vi "RemoteVI App Log Files.vi"() -> ()   [LabVIEW 2020]
doc: "Screen Log Files of RemoteVI Application Example.vi: the log files of the station (simulated - none exists on disk). Selecting a file in Log Files shows its preview and details. Delete asks in a LabVIEW dialog and removes the file from the list; Export asks for a target in the native file dialog. Runs until the notifier RemoteVI Application Example fires (the main VI quits)."
panel:
  out "Status":string
  out "Details":string
  out "Preview":dbl[][](graph)
  in  "Export":bool
  in  "Delete":bool
  in  "Log Files":i32(listbox)=-1
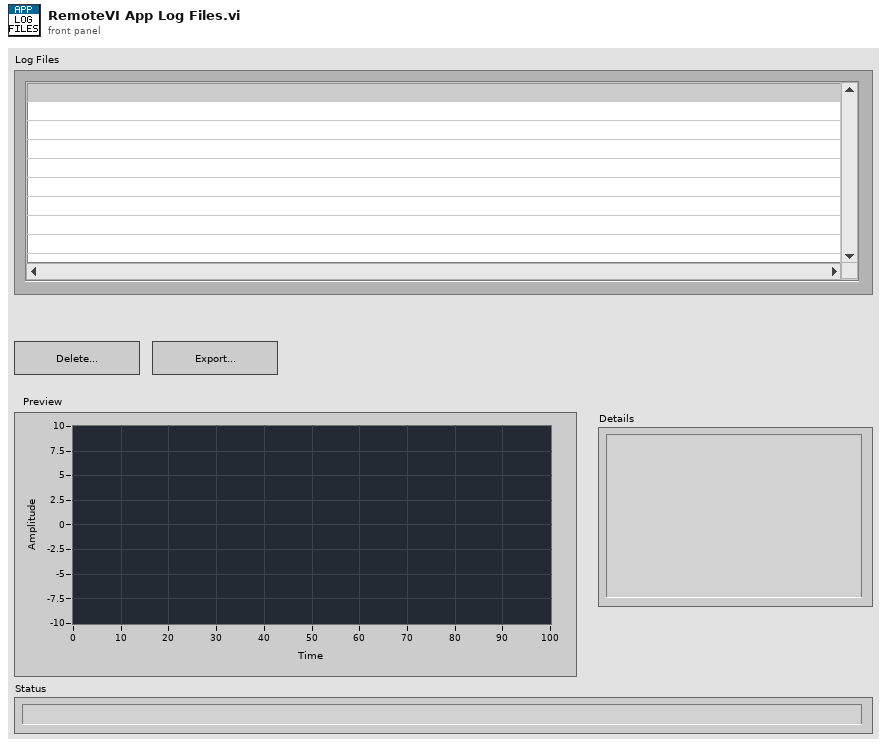
[diagram p1: front panel]
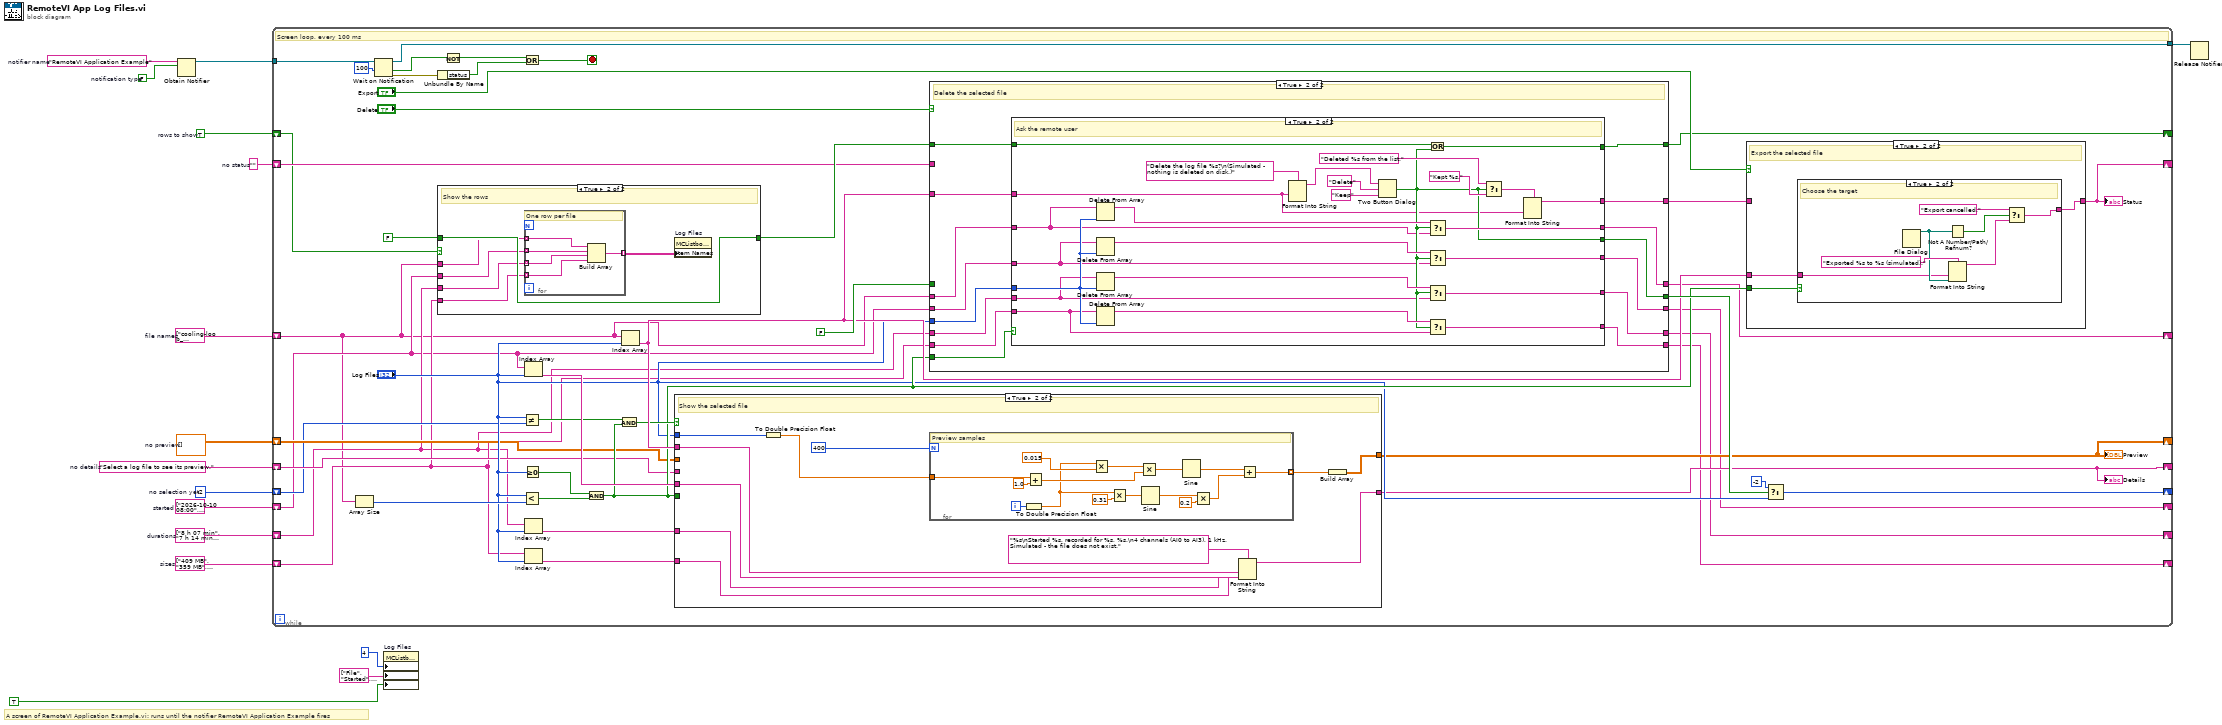
[diagram p0: block diagram]
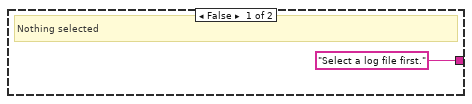
[diagram p3: hidden frame]
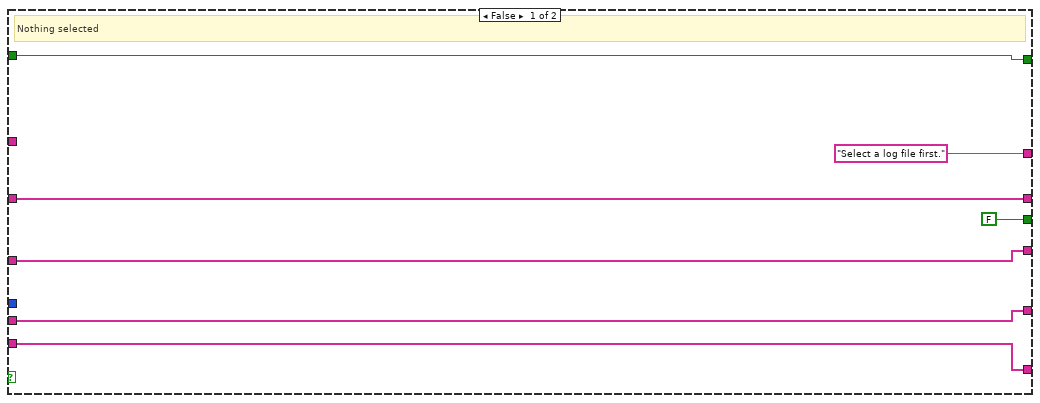
[diagram p5: hidden frame]
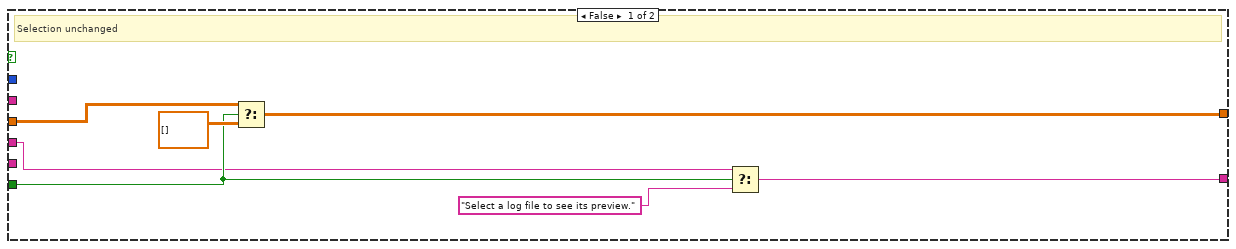
[diagram p6: hidden frame]
diagram:
  w11 = FALSE  # notification type
  w10 = "RemoteVI Application Example"  # notifier name
  w9 = ""  # no status
  w8 = "Select a log file to see its preview."  # no details
  w7 = dbl[][] []  # no preview
  w6 = -2  # no selection yet
  w5 = TRUE  # rows to show
  w4 = string[] ["409 MB", "359 MB", "411 MB", "106 MB", "413 MB", "414 MB", "364 MB", "161 MB", "417 MB", "418 MB", "419 MB", "63 MB", "421 MB", "422 MB", "423 MB", "118 MB", "374 MB", "426 MB", "427 MB", "173 MB", "429 MB"]  # sizes
  w3 = string[] ["8 h 07 min", "7 h 14 min", "8 h 21 min", "2 h 28 min", "8 h 35 min", "8 h 42 min", "7 h 49 min", "3 h 56 min", "8 h 03 min", "8 h 10 min", "8 h 17 min", "1 h 24 min", "8 h 31 min", "8 h 38 min", "8 h 45 min", "2 h 52 min", "7 h 59 min", "8 h 06 min", "8 h 13 min", "3 h 20 min", "8 h 27 min"]  # durations
  w2 = string[] ["2026-10-10 08:00", "2026-10-11 08:00", "2026-10-12 08:00", "2026-10-13 14:30", "2026-10-14 08:00", "2026-10-15 08:00", "2026-10-16 08:00", "2026-10-17 14:30", "2026-10-18 08:00", "2026-10-19 08:00", "2026-10-20 08:00", "2026-10-21 14:30", "2026-10-22 08:00", "2026-10-23 08:00", "2026-10-24 08:00", "2026-10-25 14:30", "2026-10-26 08:00", "2026-10-27 08:00", "2026-10-28 08:00", "2026-10-29 14:30", "2026-10-30 08:00"]  # started
  w1 = string[] ["cooling-loop_2026-10-10_0800.tdms", "cooling-loop_2026-10-11_0800.tdms", "cooling-loop_2026-10-12_0800.tdms", "pump-test_2026-10-13_1430.tdms", "cooling-loop_2026-10-14_0800.tdms", "cooling-loop_2026-10-15_0800.tdms", "cooling-loop_2026-10-16_0800.tdms", "pump-test_2026-10-17_1430.tdms", "cooling-loop_2026-10-18_0800.tdms", "cooling-loop_2026-10-19_0800.tdms", "cooling-loop_2026-10-20_0800.tdms", "pump-test_2026-10-21_1430.tdms", "cooling-loop_2026-10-22_0800.tdms", "cooling-loop_2026-10-23_0800.tdms", "cooling-loop_2026-10-24_0800.tdms", "pump-test_2026-10-25_1430.tdms", "cooling-loop_2026-10-26_0800.tdms", "cooling-loop_2026-10-27_0800.tdms", "cooling-loop_2026-10-28_0800.tdms", "pump-test_2026-10-29_1430.tdms", "cooling-loop_2026-10-30_0800.tdms"]  # file names
  # "A screen of RemoteVI Application Example.vi: runs until the notifier RemoteVI Application Example fires"
  n1 = Obtain Notifier(name (unnamed)=w10, notification data type=w11) -> (notifier out=w12:refnum<notifier>)  [unwired: 2 in, 2 out]
  n2 = while {
    shift-right: [w19] -> _
    shift-left: w1 -> [w18]
    shift-right: [w21] -> _
    shift-left: w2 -> [w20]
    shift-right: [w23] -> _
    shift-left: w3 -> [w22]
    shift-right: [w25] -> _
    shift-left: w4 -> [w24]
    shift-right: [w27] -> _
    shift-left: w5 -> [w26]
    shift-right: [w29] -> _
    shift-left: w6 -> [w28]
    shift-right: [w31] -> _
    shift-left: w7 -> [w30]
    shift-right: [w33] -> _
    shift-left: w8 -> [w32]
    shift-right: [w35] -> _
    shift-left: w9 -> [w34]
    tunnel: w12 -> [w17]
    tunnel: [w56] -> w16
    stop <- w61 stop-if-true
    # "Screen loop, every 100 ms"
    n3 = Array Size(array=w18) -> (size(s)=w41:i32)
    n4 = Wait on Notification(notifier=w17, timeout in ms (-1)=100) -> (notifier out=w56:refnum<notifier>, timed out?=w57:bool, error out=w58:errorcluster)  [unwired: 2 in, 1 out]
    n5 = Unbundle By Name(w58) -> ("status"=w60:bool)
    n6 = case shown="True" w26 {
      tunnel: FALSE -> [w161 w166]
      tunnel: w18 -> [_ w162]
      tunnel: w20 -> [_ w163]
      tunnel: w22 -> [_ w164]
      tunnel: w24 -> [_ w165]
      tunnel: [w161 w166] -> w40
      frame False {
        # "Rows unchanged"
      }
      frame True {
        # "Show the rows"
        n7 = for {
          tunnel: w162 -> [w168] mode=indexing
          tunnel: w163 -> [w169] mode=indexing
          tunnel: w164 -> [w170] mode=indexing
          tunnel: w165 -> [w171] mode=indexing
          tunnel: [w172] -> w167 mode=indexing
          # "One row per file"
          n8 = Build Array(w168, w169, w170, w171) -> (w172:string[])
        }
        n9 = property on="Log Files" class="MCListbox (strict)"("Item Names"=w167) -> ()  [unwired: 2 in, 2 out]
      }
    }
    n10 = Not(x=w57) -> (.not. x?=w59:bool)
    n11 = Or(x=w59, y=w60) -> (x .or. y?=w61:bool)
    n12 = Not Equal?(x="Log Files", y=w28) -> (x != y?=w45:bool)
    n13 = Less?(x="Log Files", y=w41) -> (x < y?=w43:bool)
    n14 = Greater Or Equal To 0?(x="Log Files") -> (x >= 0?=w42:bool)
    n15 = Index Array(array=w20, index="Log Files") -> (element=w48:string)
    n16 = Index Array(array=w22, index="Log Files") -> (element=w49:string)
    n17 = Index Array(array=w24, index="Log Files") -> (element=w50:string)
    n18 = And(x=w42, y=w43) -> (x .and. y?=w44:bool)
    n19 = And(x=w45, y=w44) -> (x .and. y?=w46:bool)
    n20 = Index Array(array=w18, index="Log Files") -> (element=w47:string)
    n21 = case shown="True" w46 {
      tunnel: "Log Files" -> [_ w135]
      tunnel: w30 -> [w128 _]
      tunnel: w32 -> [w129 _]
      tunnel: w47 -> [_ w136]
      tunnel: w48 -> [_ w137]
      tunnel: w49 -> [_ w138]
      tunnel: w50 -> [_ w139]
      tunnel: w44 -> [w130 _]
      tunnel: [w133 w143] -> w31
      tunnel: [w134 w145] -> w33
      frame False {
        # "Selection unchanged"
        n22 = Select(t=w128, s=w130, f=dbl[][] []) -> (s? t:f=w133:dbl[][])
        n23 = Select(t=w129, s=w130, f="Select a log file to see its preview.") -> (s? t:f=w134:string)
      }
      frame True {
        # "Show the selected file"
        n24 = To Double Precision Float(number=w135) -> (double precision float=w140:dbl)
        n25 = for {
          N: 400 -> [_]
          tunnel: w140 -> [w147]
          tunnel: [w160] -> w142 mode=indexing
          i -> [w146]
          # "Preview samples"
          n26 = To Double Precision Float(number=w146) -> (double precision float=w148:dbl)
          n27 = Add(x=w147, y=1.0) -> (x+y=w151:dbl)
          n28 = Multiply(x=w148, y=0.015) -> (x*y=w152:dbl)
          n29 = Multiply(x=w148, y=0.31) -> (x*y=w156:dbl)
          n30 = Multiply(x=w152, y=w151) -> (x*y=w153:dbl)
          n31 = Sine(x=w156) -> (sin(x)=w157:dbl)
          n32 = Sine(x=w153) -> (sin(x)=w154:dbl)
          n33 = Multiply(x=w157, y=0.2) -> (x*y=w159:dbl)
          n34 = Add(x=w154, y=w159) -> (x+y=w160:dbl)
        }
        n35 = Format Into String(format string="%s\nStarted %s, recorded for %s, %s.\n4 channels (AI0 to AI3), 1 kHz. Simulated - the file does not exist.", w136, w137, w138, w139) -> (resulting string=w145:string)  [unwired: 2 in, 1 out]
        n36 = Build Array(w142) -> (w143:dbl[][])
      }
    }
    "Preview" <- w31
    "Details" <- w33
    n37 = case shown="True" "Delete" {
      tunnel: "Log Files" -> [_ w86]
      tunnel: FALSE -> [w80 _]
      tunnel: w18 -> [w74 w81]
      tunnel: w20 -> [w75 w82]
      tunnel: w22 -> [w76 w83]
      tunnel: w24 -> [w77 w84]
      tunnel: w34 -> [w79 _]
      tunnel: [w80 w94] -> w52
      tunnel: w40 -> [w78 w85]
      tunnel: w47 -> [_ w87]
      tunnel: [w74 w89] -> w19
      tunnel: [w75 w90] -> w21
      tunnel: [w76 w91] -> w23
      tunnel: [w77 w92] -> w25
      tunnel: [w79 w95] -> w53
      tunnel: [w78 w93] -> w27
      tunnel: w44 -> [_ w88]
      frame False {
        # "Not pressed"
      }
      frame True {
        # "Delete the selected file"
        n38 = case shown="True" w88 {
          tunnel: [FALSE w114] -> w94
          tunnel: ["Select a log file first." w127] -> w95
          tunnel: w86 -> [_ w108]
          tunnel: w81 -> [w96 w103]
          tunnel: w82 -> [w97 w104]
          tunnel: w83 -> [w98 w105]
          tunnel: w84 -> [w99 w106]
          tunnel: w85 -> [w100 w107]
          tunnel: w87 -> [_ w109]
          tunnel: [w96 w116] -> w89
          tunnel: [w97 w118] -> w90
          tunnel: [w98 w120] -> w91
          tunnel: [w99 w122] -> w92
          tunnel: [w100 w123] -> w93
          frame False {
            # "Nothing selected"
          }
          frame True {
            # "Ask the remote user"
            n39 = Delete From Array(array=w103, index=w108) -> (array with subset deleted=w115:string[])  [unwired: 1 in, 1 out]
            n40 = Delete From Array(array=w104, index=w108) -> (array with subset deleted=w117:string[])  [unwired: 1 in, 1 out]
            n41 = Delete From Array(array=w105, index=w108) -> (array with subset deleted=w119:string[])  [unwired: 1 in, 1 out]
            n42 = Delete From Array(array=w106, index=w108) -> (array with subset deleted=w121:string[])  [unwired: 1 in, 1 out]
            n43 = Format Into String(format string="Delete the log file %s?\n(Simulated - nothing is deleted on disk.)", w109) -> (resulting string=w111:string)  [unwired: 2 in, 1 out]
            n44 = Two Button Dialog(message=w111, 1:"Keep", 2:"Delete") -> (T button?=w114:bool)
            n45 = Or(x=w107, y=w114) -> (x .or. y?=w123:bool)
            n46 = Select(t=w115, s=w114, f=w103) -> (s? t:f=w116:string[])
            n47 = Select(t=w117, s=w114, f=w104) -> (s? t:f=w118:string[])
            n48 = Select(t=w119, s=w114, f=w105) -> (s? t:f=w120:string[])
            n49 = Select(t=w121, s=w114, f=w106) -> (s? t:f=w122:string[])
            n50 = Select(t="Deleted %s from the list.", s=w114, f="Kept %s.") -> (s? t:f=w126:string)
            n51 = Format Into String(format string=w126, w109) -> (resulting string=w127:string)  [unwired: 2 in, 1 out]
          }
        }
      }
    }
    n52 = case shown="True" "Export" {
      tunnel: w47 -> [_ w63]
      tunnel: w53 -> [w62 _]
      tunnel: w44 -> [_ w64]
      tunnel: [w62 w65] -> w35
      frame False {
        # "Not pressed"
      }
      frame True {
        # "Export the selected file"
        n53 = case shown="True" w64 {
          tunnel: ["Select a log file first." w73] -> w65
          tunnel: w63 -> [_ w67]
          frame False {
            # "Nothing selected"
          }
          frame True {
            # "Choose the target"
            n54 = File Dialog() -> (3:w68:path)  [unwired: 7 in, 3 out]
            n55 = Not A Number/Path/Refnum?(number/path/refnum=w68) -> (NaN/Path/Refnum?=w69:bool)
            n56 = Format Into String(format string="Exported %s to %s (simulated).", w67, w68) -> (resulting string=w71:string)  [unwired: 2 in, 1 out]
            n57 = Select(t="Export cancelled.", s=w69, f=w71) -> (s? t:f=w73:string)
          }
        }
      }
    }
    "Status" <- w35
    n58 = Select(t=-2, s=w52, f="Log Files") -> (s? t:f=w29:i32)
  }
  n59 = property on="Log Files" class="MCListbox (strict)"("Number of Columns"=4, "Column Header Strings[]"=string[] ["File", "Started", "Duration", "Size"], "Visible Items:Column Headers Visible"=TRUE) -> ()  [unwired: 2 in, 2 out]
  n60 = Release Notifier(notifier=w16) -> ()  [unwired: 2 in, 3 out]
